vi "CLI Demo.vi"() -> ()   [LabVIEW 2015]
doc: "Demo application for the G-CLI"
uses:
  CLI Class/CLI.lvclass
panel:
  in  "Path":path
  in  "Send File":bool
  in  "Exit Error":errorcluster
  in  "Length (chars)":i32=2048
  in  "Send Random":bool
  out "CLI Input Arguments":string[](array[string])
  in  "stop":bool
  in  "Send Line":bool
  in  "Line":string
  # "To try out the CLI tool. Call this VI from the command line. The exact path depends on your LabVIEW version.\n\nPress Ctrl+I and look under the general tab to get the path."
  # "Writes a single line to the command line."
  # "Writes a large random string to the command line."
  # "Writes the contents of a text file to the command line."
  # "When you stop - the exit error will define the return code."
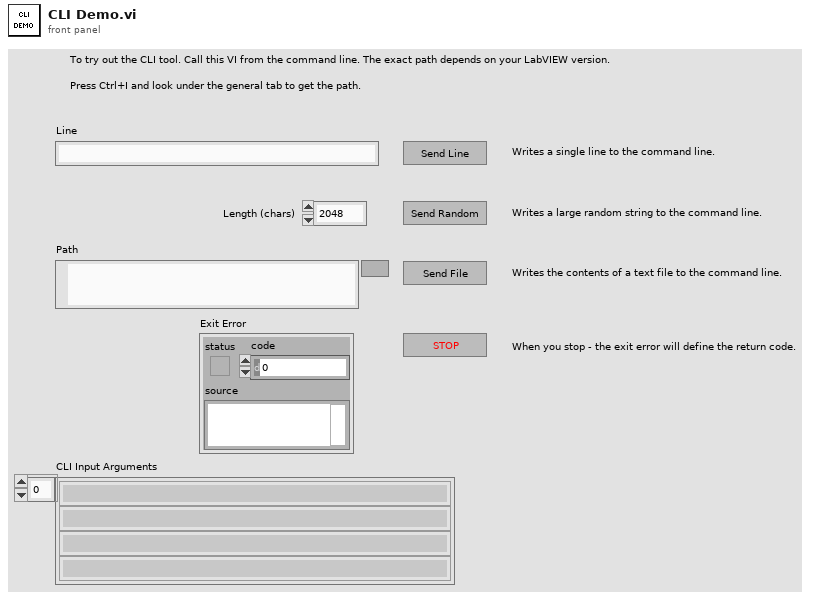
[diagram p1: front panel]
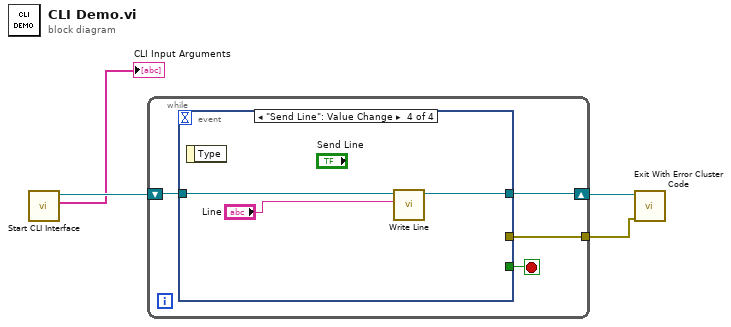
[diagram p0: block diagram]
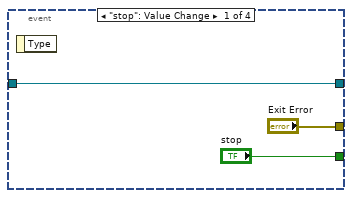
[diagram p2: hidden frame]
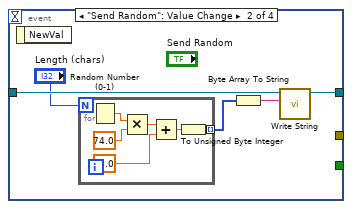
[diagram p3: hidden frame]
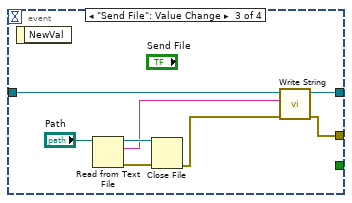
[diagram p4: hidden frame]
diagram:
  n1 = call "Start CLI Interface.vi"() -> ("Custom Parameters"=→"CLI Input Arguments":string[], "CLI out"=w4:refnum<class "CLI.lvclass">)  [unwired: 8 in, 2 out]
  n2 = while {
    shift-right: [w7] -> w3
    shift-left: w4 -> [w6]
    tunnel: [w5] -> w1
    stop <- w8 stop-if-true
    n3 = event shown="[3] \"Send Line\": Value Change" {
      selector: _ -> [_ _ _ _]
      dyn-events: _ -> [_ _ _ _]
      timeout: _ -> [_ _ _ _]
      tunnel: ["stop" _ _ _] -> w8
      tunnel: [w10 w16 w30 w33] -> w7
      tunnel: w6 -> [w10 w15 w29 w32]
      tunnel: ["Exit Error" _ w24 _] -> w5
      event "stop": Value Change {
        n4 = event-data() -> ()  [unwired: 1 in, 1 out]
      }
      event "Send Random": Value Change {
        n5 = event-data() -> ()  [unwired: 1 in, 1 out]
        n6 = for {
          N: "Length (chars)" -> [_]
          tunnel: [w17] -> w13 mode=indexing
          n7 = Random Number (0-1)() -> (number: 0 to 1=w18:dbl)
          n8 = Multiply(x=w18, y=74.0) -> (x*y=w20:dbl)
          n9 = Add(x=w20, y=48.0) -> (x+y=w22:dbl)
          n10 = To Unsigned Byte Integer(number=w22) -> (unsigned 8bit integer=w17:u8)
        }
        n11 = Byte Array To String(unsigned byte array=w13) -> (string=w12:string)
        n12 = call "Write String.vi"("Text to Write"=w12, "CLI in"=w15) -> ("CLI out"=w16:refnum<class "CLI.lvclass">)  [unwired: 8 in, 1 out]
      }
      event "Send File": Value Change {
        n13 = event-data() -> ()  [unwired: 1 in, 1 out]
        n14 = Read from Text File(file (use dialog)="Path") -> (refnum out=w26:refnum<file>, text=w23:string, error out=w27:errorcluster)  [unwired: 3 in, 1 out]
        n15 = Close File(refnum=w26, error in=w27) -> (error out=w25:errorcluster)  [unwired: 1 out]
        n16 = call "Write String.vi"("error in (no error)"=w25, "Text to Write"=w23, "CLI in"=w29) -> ("error out"=w24:errorcluster, "CLI out"=w30:refnum<class "CLI.lvclass">)  [unwired: 7 in]
      }
      event "Send Line": Value Change {
        n17 = event-data() -> ()  [unwired: 1 in, 1 out]
        n18 = call "Write Line.vi"("Text to Write"="Line", "CLI in"=w32) -> ("CLI out"=w33:refnum<class "CLI.lvclass">)  [unwired: 8 in, 1 out]
      }
    }
  }
  n19 = call "Exit With Error Cluster Code.vi"("error in (no error)"=w1, "CLI in"=w3) -> ()  [unwired: 9 in, 1 out]
